vi "Regulation - Interpolate and Measure.vi"(0 "measurement configuration":T7 {"acq sampling rate" format="%0.2f"; "master clock rate" format="%#_6pHz"; "frame clock rate" format="%#_6pHz"}, 2 "regulation settings":T3={"enable regulation"=FALSE, "regulation target"=enum."THD+N Ratio", "regulation target value"=0.05, "regulation target value units"=enum."%", "regulation start level"=10.0, "regulation stop level"=70.0, "regulation number of steps"=2}, 3 "search results":cluster{"level":dbl, "value":dbl}[](array[cluster]), 5 "error in (no error)":errorcluster, 7 "PCM tasks":T1, 9 "DAQmx task in":refnum<k21>) -> (11 "PCM tasks":T1, 13 "DAQmx task out":refnum<k21>, 14 "results":T6, 16 "time domain":waveform(dbl), 17 "spectrum":cluster{"x0":dbl, "dx":dbl, "magnitude":dbl[]}, 18 "output power":dbl, 19 "error out":errorcluster)   [LabVIEW 2021]
uses:
  controls/single tone measurement settings (HW).ctl
  controls/digital audio protocol/data justification.ctl
  controls/digital audio protocol/endianness.ctl
  controls/digital audio protocol/digital edge.ctl
  controls/digital audio protocol/logic level.ctl
  controls/digital output level units.ctl
  controls/weighting filter.ctl
  controls/highpass filter.ctl
  controls/lowpass filter.ctl
  controls/units - snr.ctl
  controls/units - ratio.ctl
  controls/single tone audio measurements.ctl
  controls/regulation settings.ctl
  controls/regulation target.ctl
  controls/regulation target value units.ctl
  controls/digital audio protocol/PCM tasks.ctl
  <vilib>/PDM Acquisition Toolkit/host/Classes/Tasks/PCM Output/Controls/PCM Output Task DVR.ctl
  <vilib>/PDM Acquisition Toolkit/host/Classes/Tasks/PCM Output/PCM Output Task.lvclass
  <vilib>/gmath/NI_Gmath.lvlib
  controls/audio controls.lvlib
panel:
  out "interpolation value":dbl
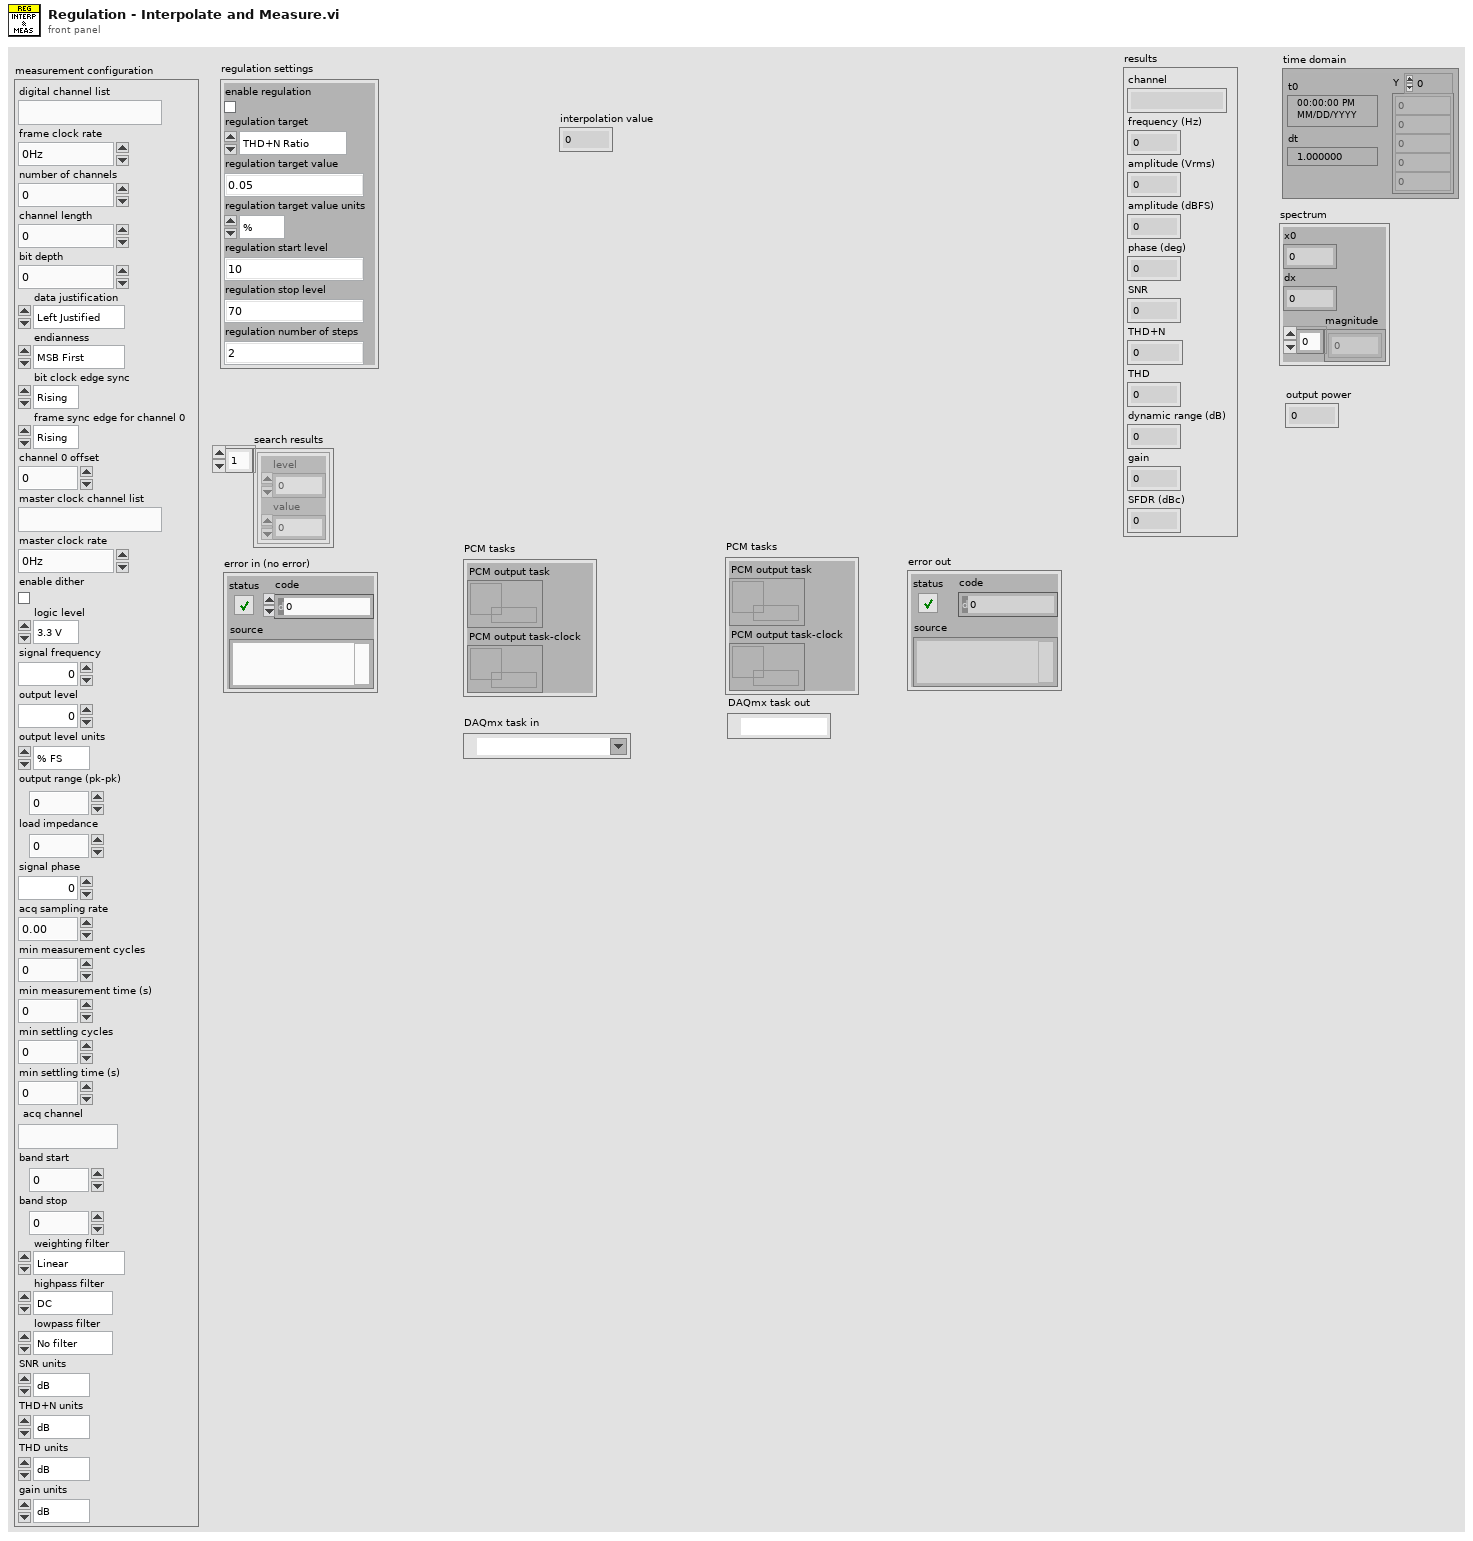
[diagram p1: front panel]
types:
  T1 = typedef "PCM tasks.ctl" = cluster{"PCM output task":T2, "PCM output task-clock":T2}
  T2 = typedef "PDM Acquisition Class Library.lvlib/PCM Output Task.lvclass/PCM Output Task DVR.ctl" = refnum<data-value>
  T3 = typedef "regulation settings.ctl" = cluster{"enable regulation":bool, "regulation target":T4, "regulation target value":dbl, "regulation target value units":T5, "regulation start level":dbl, "regulation stop level":dbl, "regulation number of steps":u32}
  T4 = typedef "regulation target.ctl" = enum32{"THD+N Ratio", "Output Power"}
  T5 = typedef "regulation target value units.ctl" = enum32{"%", "W"}
  T6 = typedef "audio controls.lvlib/single tone audio measurements.ctl" = cluster{"channel":string, "frequency (Hz)":dbl, "amplitude (Vrms)":dbl, "amplitude (dBFS)":dbl, "phase (deg)":dbl, "SNR":dbl, "THD+N":dbl, "THD":dbl, "dynamic range (dB)":dbl, "gain":dbl, "SFDR (dBc)":dbl}
  T7 = typedef "single tone measurement settings (HW).ctl" = cluster{"digital channel list":string, "frame clock rate":dbl, "number of channels":u32, "channel length":u32, "bit depth":u32, "data justification":T8, "endianness":T9, "bit clock edge sync":T10, "frame sync edge for channel 0":T10, "channel 0 offset":u32, "master clock channel list":string, "master clock rate":dbl, "enable dither":bool, "logic level":T11, "signal frequency":dbl, "output level":dbl, "output level units":T12, "output range (pk-pk)":dbl, "load impedance":dbl, "signal phase":dbl, "acq sampling rate":dbl, "min measurement cycles":u32, "min measurement time (s)":dbl, "min settling cycles":u32, "min settling time (s)":dbl, "acq channel":string, "band start":dbl, "band stop":dbl, "weighting filter":T13, "highpass filter":T14, "lowpass filter":T15, "SNR units":T16, "THD+N units":T17, "THD units":T17, "gain units":T17}
  T8 = typedef "data justification.ctl" = enum32{"Left Justified", "Right Justified"}
  T9 = typedef "endianness.ctl" = enum32{"MSB First", "LSB First"}
  T10 = typedef "digital edge.ctl" = enum32{"Rising", "Falling"}
  T11 = typedef "logic level.ctl" = enum32{"3.3 V", "1.8 V", "1.2 V"}
  T12 = typedef "audio controls.lvlib/digital output level units.ctl" = enum32{"% FS", "dBFS", "V"}
  T13 = typedef "weighting filter.ctl" = enum32{"Linear", "A-weighting", "B-weighting", "C-weighting"}
  T14 = typedef "highpass filter.ctl" = enum32{"DC", "AC"}
  T15 = typedef "lowpass filter.ctl" = enum32{"No filter", "AES17 20kHz", "AES17 40kHz"}
  T16 = typedef "audio controls.lvlib/units - snr.ctl" = enum32{"dB", "x/y"}
  T17 = typedef "audio controls.lvlib/units - ratio.ctl" = enum32{"dB", "%", "x/y"}
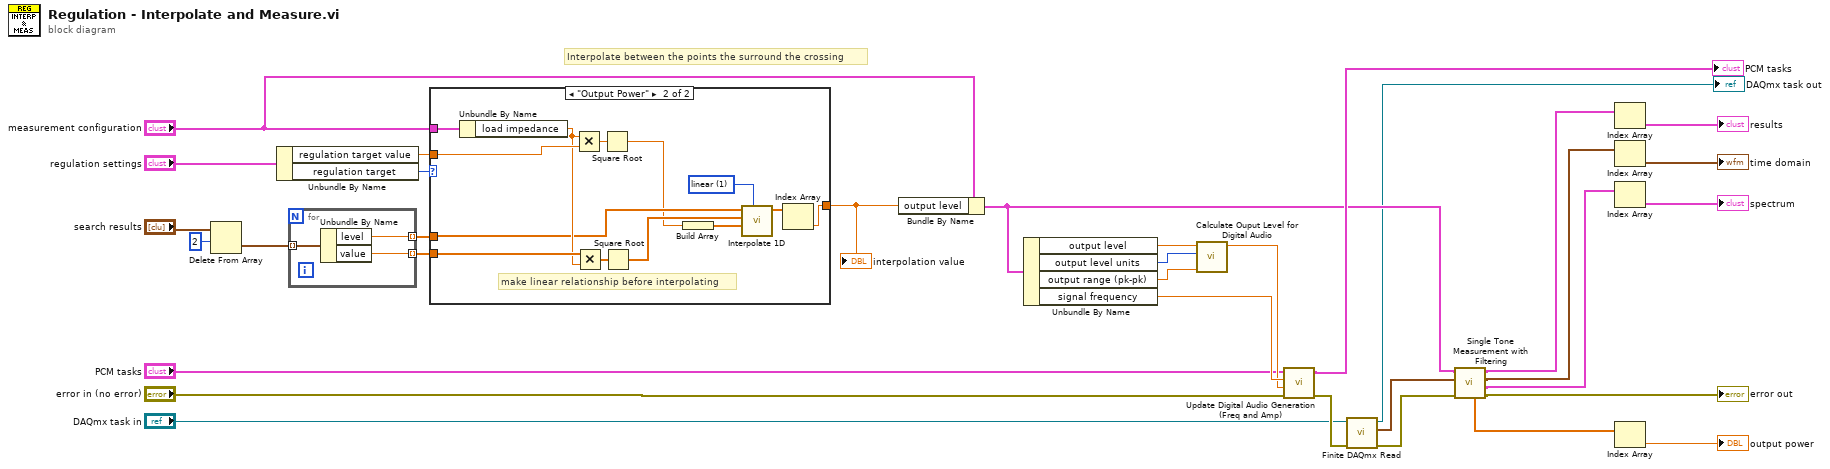
[diagram p0: block diagram]
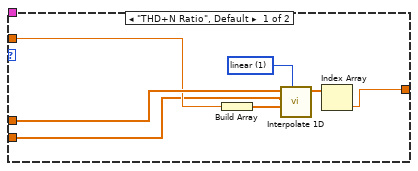
[diagram p2: hidden frame]
diagram:
  # "Interpolate between the points the surround the crossing"
  n1 = Delete From Array(array="search results", length=2) -> (deleted portion=w25:cluster{"level":dbl, "value":dbl}[])  [unwired: 1 in, 1 out]
  n2 = Unbundle By Name("regulation settings") -> ("regulation target value"=w32:dbl, "regulation target"=w30:T4)
  n3 = for {
    tunnel: w25 -> [w36] mode=indexing
    tunnel: [w35] -> w28 mode=indexing
    tunnel: [w34] -> w29 mode=indexing
    n4 = Unbundle By Name(w36) -> ("level"=w34:dbl, "value"=w35:dbl)
  }
  n5 = case shown="\"Output Power\"" w30 {
    tunnel: w32 -> [w39 w52]
    tunnel: [w41 w44] -> w31
    tunnel: w29 -> [w40 w50]
    tunnel: w28 -> [w37 w53]
    tunnel: "measurement configuration" -> [_ w56]
    frame "THD+N Ratio", Default {
      w43 = 1 items=["nearest", "linear", "spline", "cubic Hermite", "Lagrange"] ("method")
      n6 = Build Array(w39) -> (w38:dbl[])
      n7 = call <vilib>:"Interpolate 1D.vi"("method"=w43, "xi"=w38, "X"=w37, "Y"=w40) -> ("yi"=w42:dbl[])  [unwired: 5 in, 2 out]
      n8 = Index Array(array=w42) -> (element=w41:dbl)  [unwired: 1 in]
    }
    frame "Output Power" {
      w46 = 1 items=["nearest", "linear", "spline", "cubic Hermite", "Lagrange"] ("method")
      # "make linear relationship before interpolating"
      n9 = Unbundle By Name(w56) -> ("load impedance"=w51:dbl)
      n10 = Multiply(x=w51, y=w52) -> (x*y=w55:dbl)
      n11 = Multiply(x=w53, y=w51) -> (x*y=w54:dbl[])
      n12 = Square Root(x=w55) -> (sqrt(x)=w48:dbl)
      n13 = Square Root(x=w54) -> (sqrt(x)=w49:dbl[])
      n14 = Build Array(w48) -> (w47:dbl[])
      n15 = call <vilib>:"Interpolate 1D.vi"("method"=w46, "xi"=w47, "X"=w49, "Y"=w50) -> ("yi"=w45:dbl[])  [unwired: 5 in, 2 out]
      n16 = Index Array(array=w45) -> (element=w44:dbl)  [unwired: 1 in]
    }
  }
  "interpolation value" <- w31
  n17 = Bundle By Name(cluster="measurement configuration", "output level"=w31) -> (w6:T7)
  n18 = Unbundle By Name(w6) -> ("output level"=w9:dbl, "output level units"=w8:T12, "output range (pk-pk)"=w7:dbl, "signal frequency"=w5:dbl)
  n19 = call "Calculate Ouput Level for Digital Audio.vi"("output range (pk-pk)"=w7, "digital output level units"=w8, "output level"=w9) -> ("gain"=w4:dbl)  [unwired: 7 in, 1 out]
  n20 = call "Update Digital Audio Generation (Freq and Amp).vi"("error in (no error)"="error in (no error)", "gain"=w4, "frequency"=w5, "PCM tasks"="PCM tasks") -> ("error out"=w19:errorcluster, "PCM tasks"=→"PCM tasks":T1)  [unwired: 6 in]
  n21 = call "Finite DAQmx Read.vi"("error in (no error)"=w19, "task/channels in"="DAQmx task in") -> ("error out"=w18:errorcluster, "data"=w17:waveform(dbl)[], "task out"=→"DAQmx task out":refnum<k21>)  [unwired: 7 in]
  n22 = call "Single Tone Measurement with Filtering.vi"("error in (no error)"=w18, "waveforms"=w17, "measurement configuration"=w6) -> ("error out"=→"error out":errorcluster, "spectra"=w13:cluster{"x0":dbl, "dx":dbl, "magnitude":dbl[]}[], "waveforms"=w12:waveform(dbl)[], "results"=w11:T6[], "output power"=w14:dbl[])  [unwired: 4 in]
  n23 = Index Array(array=w11) -> (element=→"results":T6)  [unwired: 1 in]
  n24 = Index Array(array=w12) -> (element=→"time domain":waveform(dbl))  [unwired: 1 in]
  n25 = Index Array(array=w13) -> (element=→"spectrum":cluster{"x0":dbl, "dx":dbl, "magnitude":dbl[]})  [unwired: 1 in]
  n26 = Index Array(array=w14) -> (element=→"output power":dbl)  [unwired: 1 in]
